vi "Measurement UI.vi"() -> ()   [LabVIEW 2025, in "I2C Bus Monitor UI.lvlib"]
uses:
  I2C Bus Monitor UI.lvlib
  OOB gRPC Client/RPC Messages/hwval_GenericRequest.ctl
  042a6803-d82a-4003-9d1e-a547103779a0.vi
  SubVIs/Table Buffer - Check.vi
  SubVIs/Table Buffer - Create.vi
  SubVIs/Table Buffer - Destroy.vi
  OOB gRPC Client/OOB gRPC Client.lvlib
panel:
  in  "HELP":bool
  in  "CMPLX SCRIPT":bool
  out "RUNNING":bool
  in  "Monitor Tab":enum32{"Monitor", "Scan"}(tab)
  out "# TXNS IN TABLE":i32
  in  "PauseResume":bool=TRUE
  out "STREAMING":bool
  in  "CSV FILE PATH":path
  in  "Save CSV":bool
  out "# TXNS IN BUFFER":i32
  in  "Clear":bool
  out "MONITOR TABLE":string[][](table)
  in  "Scan Bus":bool
  out "Scan Table":string[][](table)
  out "BUSY":bool
  in  "Debug&Hidden":enum32{"Debug", "Hidden"}(tab)
  out "Message Buffer Pressure (Logic)":i32
  out "Transactions in Buffer (UI)":i32
  out "FIFO Overflow":bool
  out "FIFO Pressure":u32
  out "Measurement Logic Counter":i32
  out "FIFO Msg Fetch Count":i32
  out "OOB gRPC Port":i32
  in  "Bitfile Path":string
  in  "Alias Name":string
  in  "Serial Input":string
  out "Error (Logic)":string
  out "Scanned Addresses":i32[](array[numeric]) format="%.0x"
  out "Status":string
  in  "Send I2C CMD":bool
  in  "R/W":bool
  in  "DATA":u8 format="%02x"
  in  "REG. ADDR.":u16 format="%04x"
  in  "SLAVE ADDR.":u8 format="%02x"
  in  "Send I2C Script":bool
  in  "CONFIG SCRIPT FILE PATH":path
  in  "SERIAL INPUT (SI)":u32(ring)
  in  "RESOURCE NAME":u32(ring)
  # "NOTE:\nFlat Box sizes are specifically chosen to fit into IS small panel without a horizontal scrollbar"
  # "CONFIGURATION"
  # "I2C TRANSACTIONS"
  # "I2C MONITOR"
  # "STATUS"
  # "These controls are mainly used to transfer data from logic to ui via configs/results, but don't need to be visible."
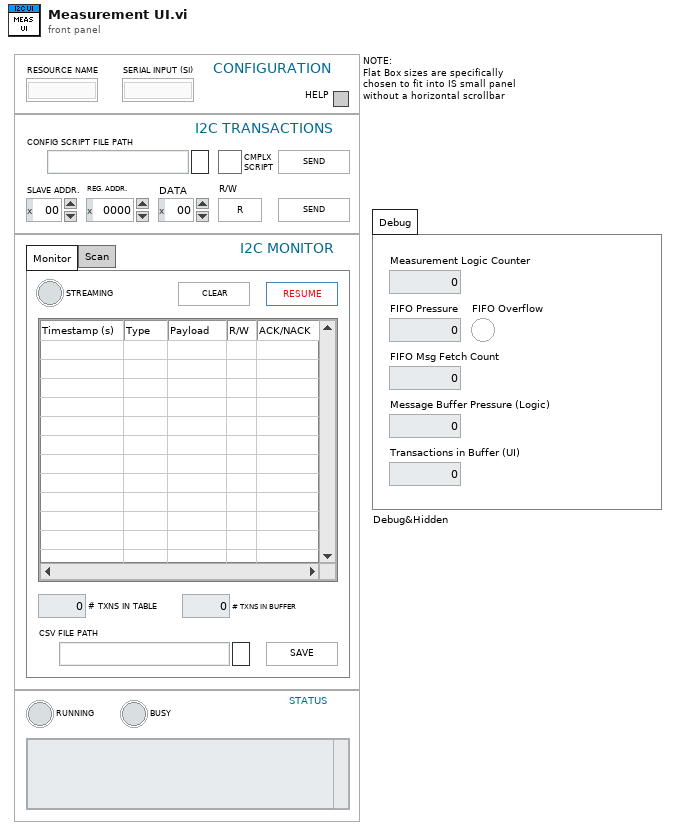
[diagram p1: front panel]
types:
  T1 = cluster{"Measurement Logic Counter":refnum<vi>, "OOB gRPC Port":refnum<vi>, "Bitfile Path":refnum<vi>, "RESOURCE NAME":refnum<vi>, "Alias Name":refnum<vi>, "SERIAL INPUT (SI)":refnum<vi>, "Serial Input":refnum<vi>, "MONITOR TABLE":refnum<vi>, "FIFO Msg Fetch Count":refnum<vi>, "STREAMING":refnum<vi>, "PauseResume":refnum<vi>, "Transactions in Buffer (UI)":refnum<vi>, "CSV FILE PATH":refnum<vi>, "BUSY":refnum<vi>, "Status":refnum<vi>, "Error (Logic)":refnum<vi>, "Scan Table":refnum<vi>, "Scanned Addresses":refnum<vi>, "# TXNS IN BUFFER":refnum<vi>, "# TXNS IN TABLE":refnum<vi>, "RUNNING":refnum<vi>}
  T2 = typedef "OOB gRPC Client.lvlib/hwval_GenericRequest.ctl" = cluster{"Command":string, "Payload":u8[]}
  T3 = typedef "OOB gRPC Client.lvlib/hwval_GenericResponse.ctl" = cluster{"Payload":u8[]}
  T4 = typedef "grpc-lvsupport-release.lvlib/grpcId.ctl" = u64
  T5 = cluster{"NewVal":bool, string, "CMPLX SCRIPT":bool}
  T6 = cluster{"NewVal":bool, "SLAVE ADDR.":u8, "REG. ADDR.":u16, "DATA":u8, "R/W":bool}
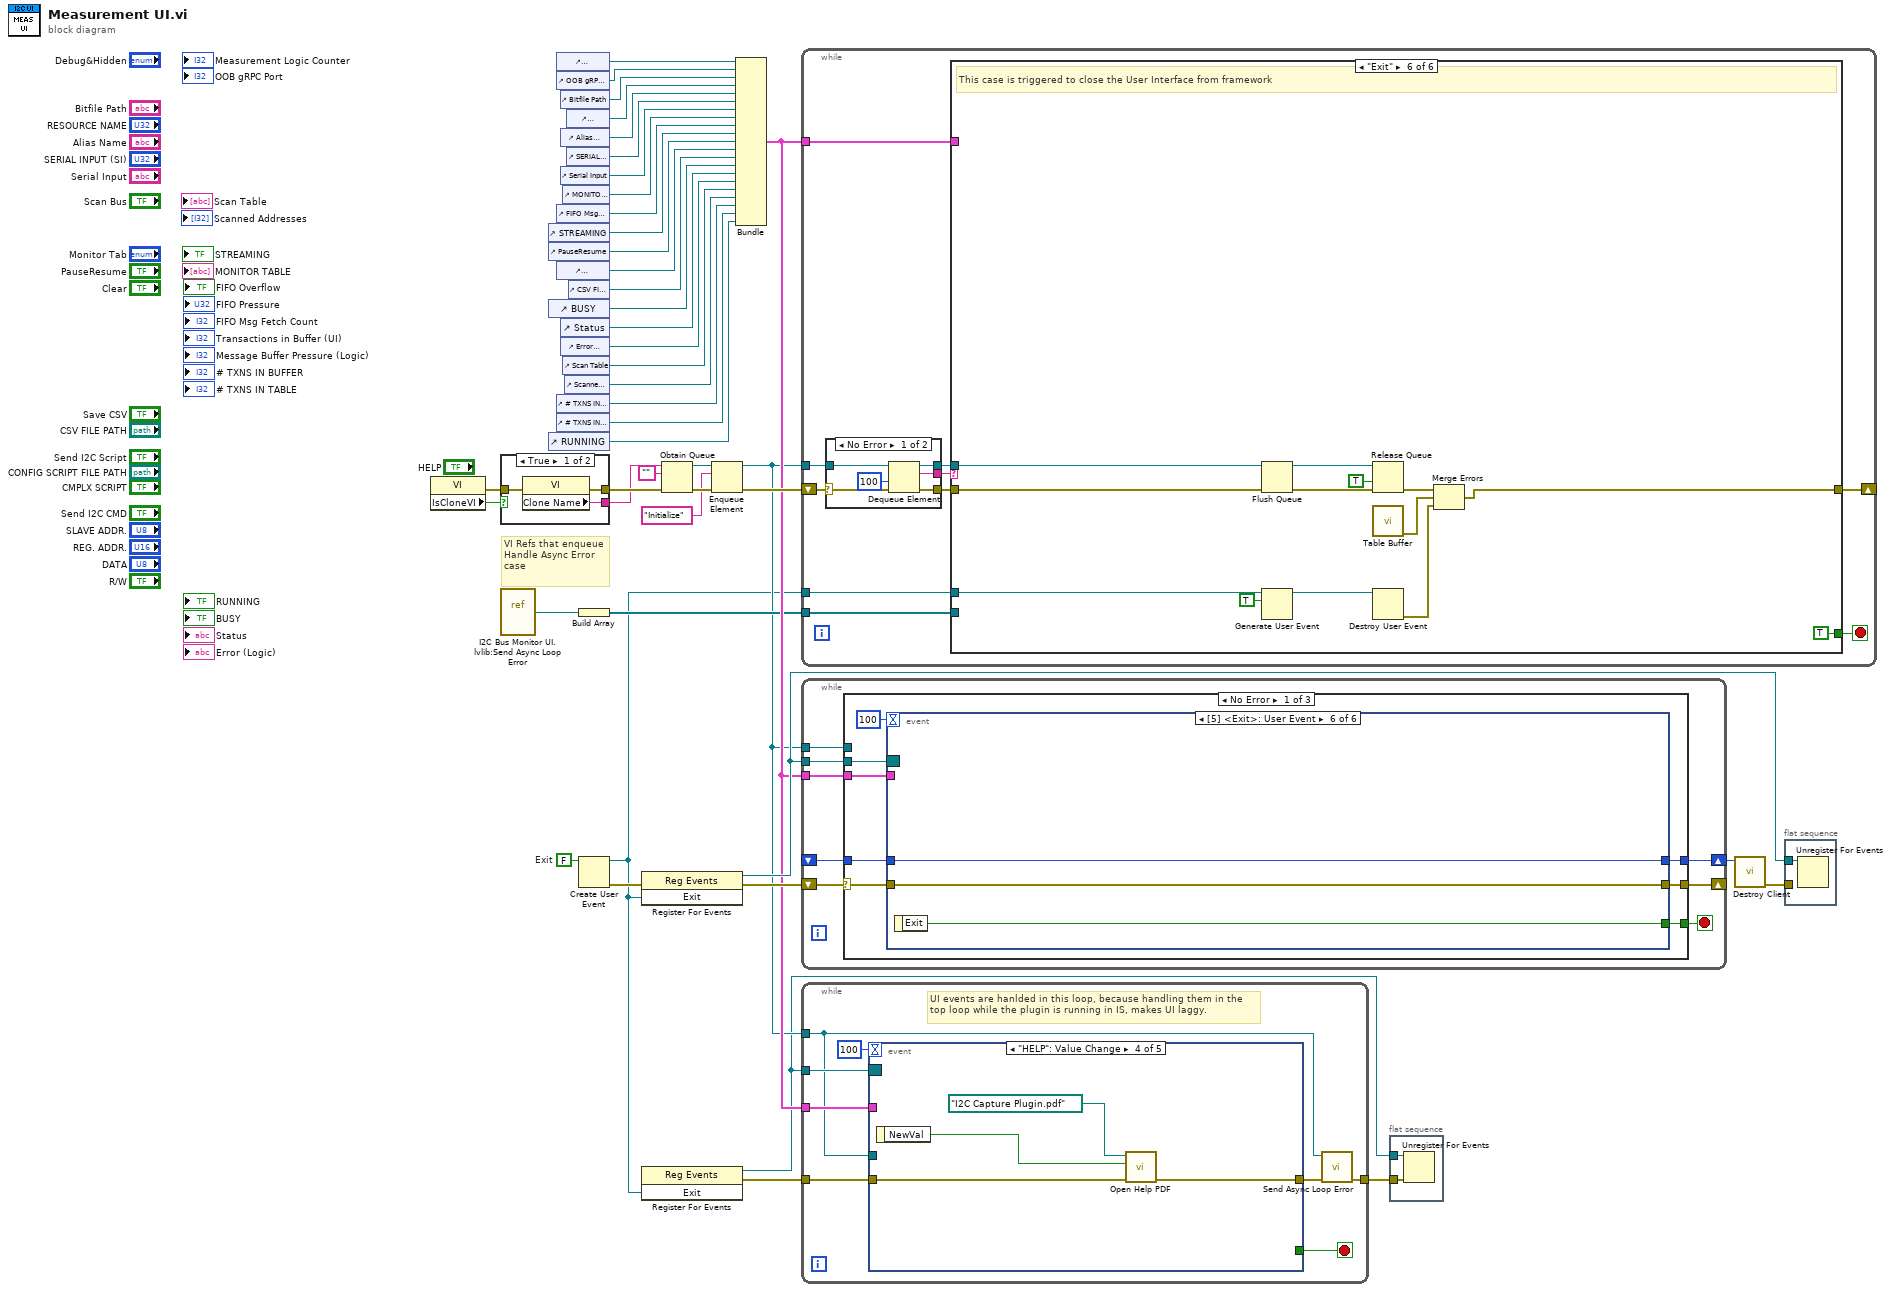
[diagram p0: block diagram]
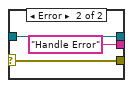
[diagram p2: hidden frame]
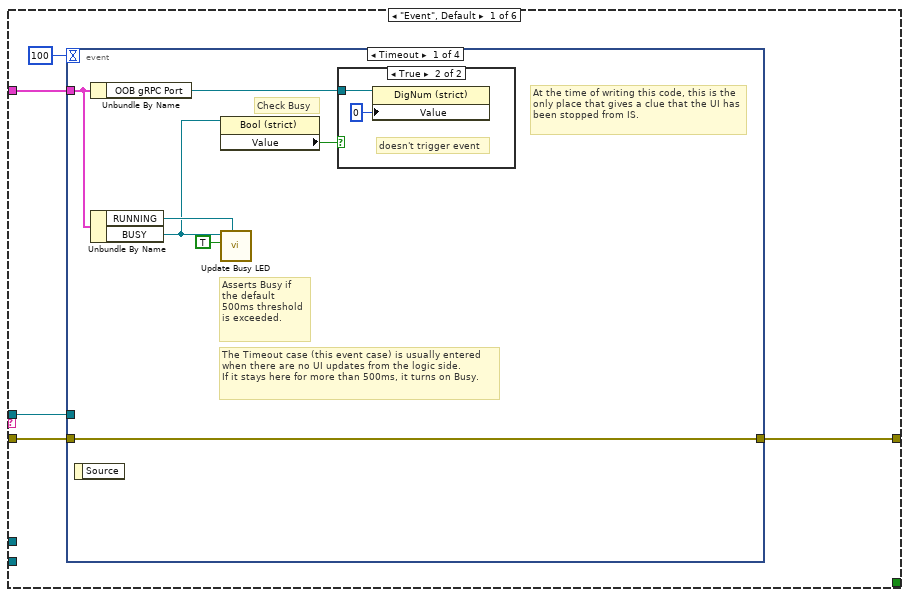
[diagram p3: hidden frame]
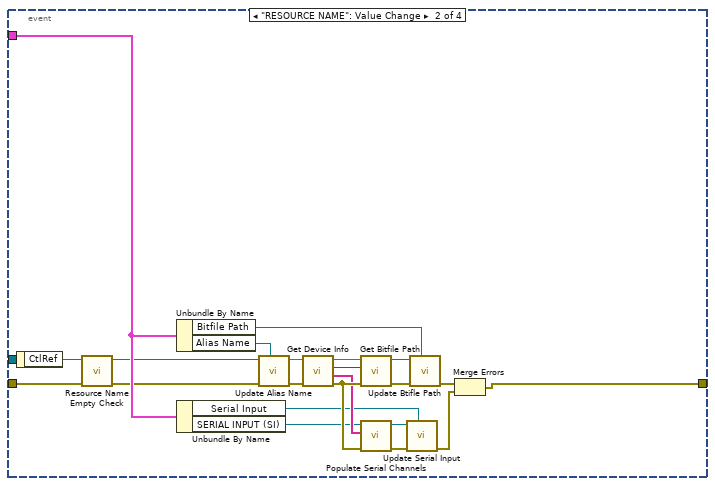
[diagram p5: hidden frame]
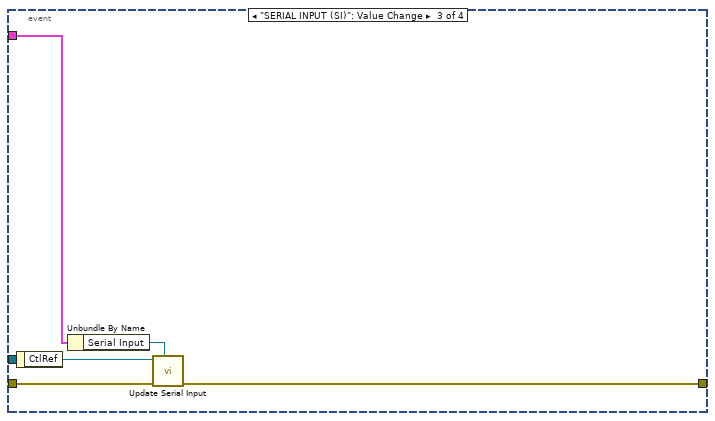
[diagram p6: hidden frame]
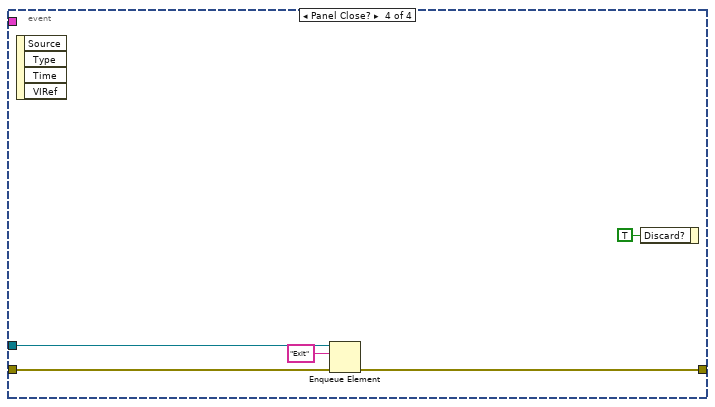
[diagram p7: hidden frame]
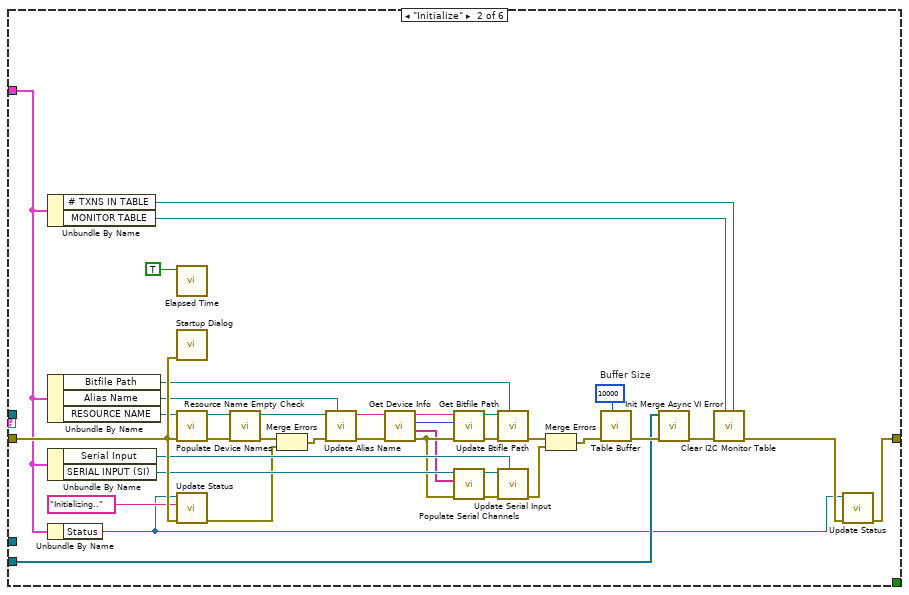
[diagram p8: hidden frame]
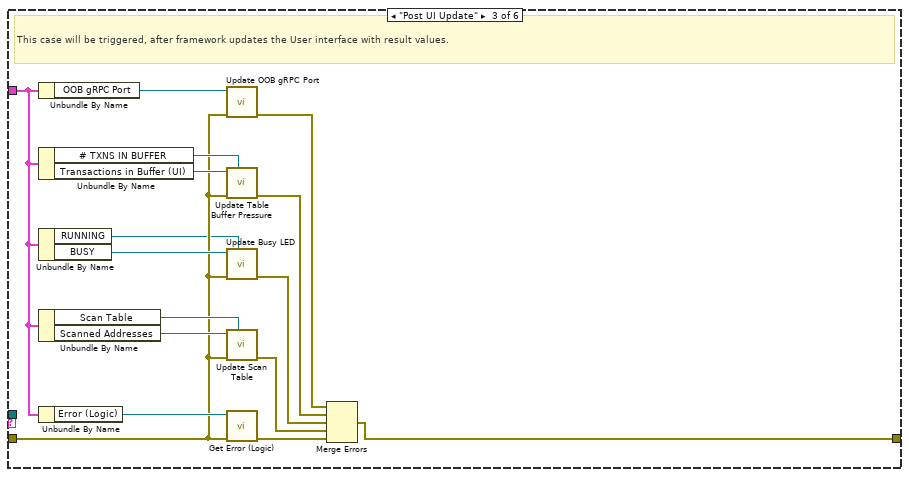
[diagram p9: hidden frame]
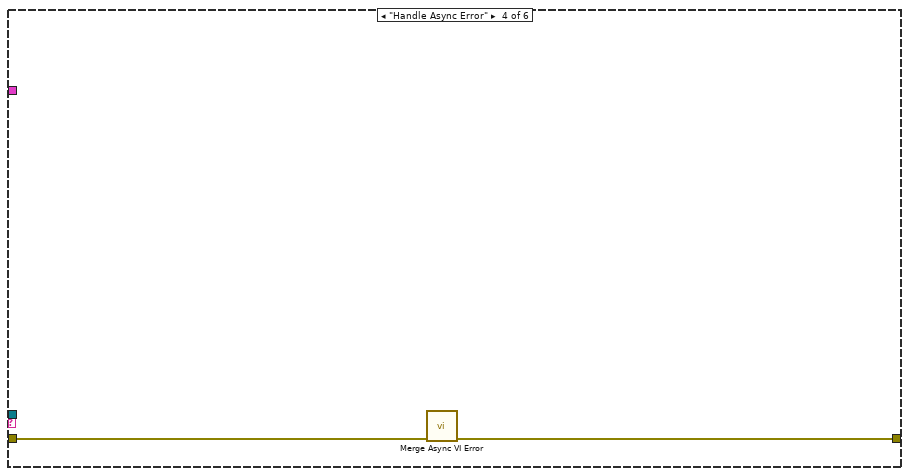
[diagram p10: hidden frame]
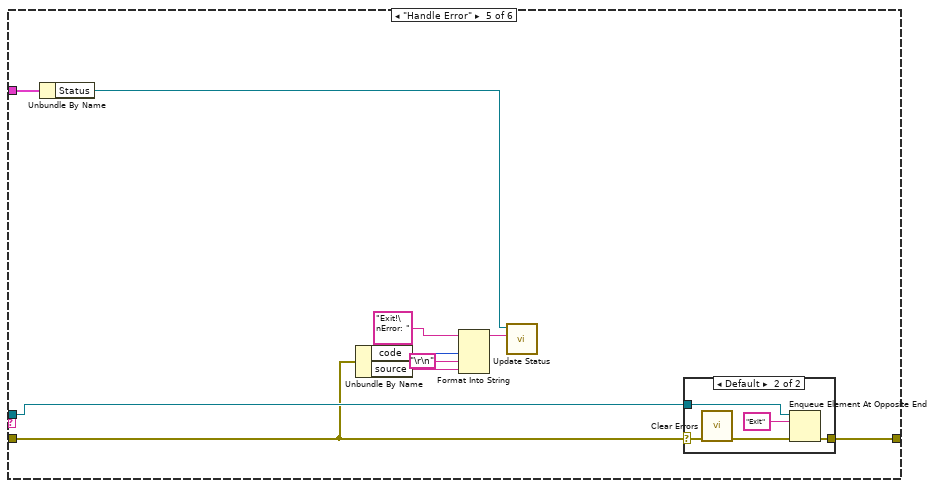
[diagram p11: hidden frame]
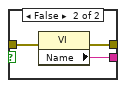
[diagram p13: hidden frame]
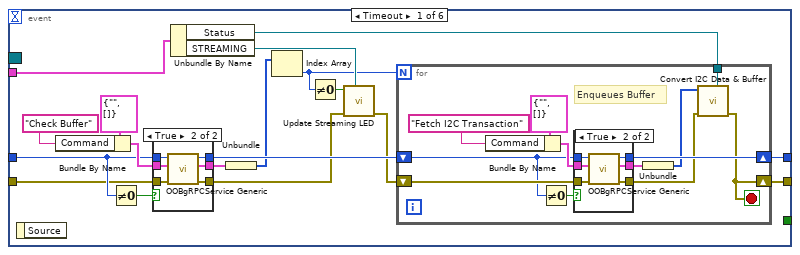
[diagram p14: hidden frame]
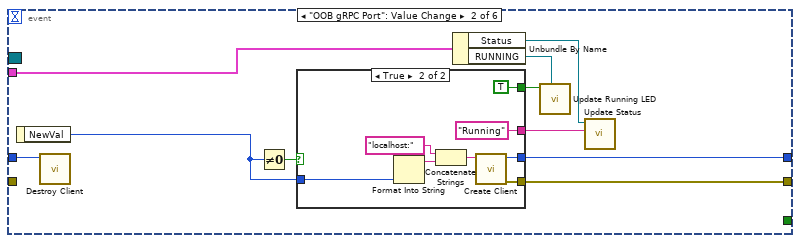
[diagram p17: hidden frame]
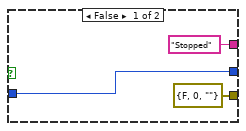
[diagram p18: hidden frame]
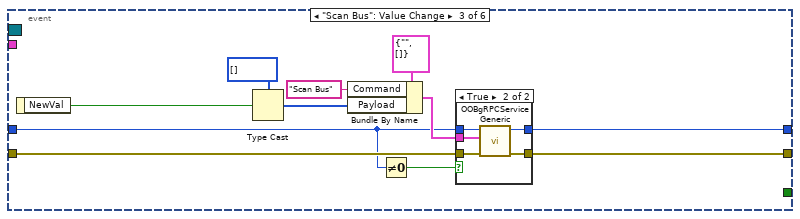
[diagram p19: hidden frame]
diagram:
  w35 = FALSE  # Exit
  # "VI Refs that enqueue Handle Async Error case"
  n1 = property class="VI"() -> (error out=w32:errorcluster, "IsCloneVI"=w36:bool)  [unwired: 2 in, 1 out]
  n2 = case shown="True" w36 {
    tunnel: [w47 w50] -> w43
    tunnel: [w46 w49] -> w42
    tunnel: w32 -> [w45 w48]
    frame True {
      n3 = property class="VI"(error in=w45) -> (error out=w47:errorcluster, "Clone Name"=w46:string)  [unwired: 1 in, 1 out]
    }
    frame False {
      n4 = property class="VI"(error in=w48) -> (error out=w50:errorcluster, "Name"=w49:string)  [unwired: 1 in, 1 out]
    }
  }
  n5 = vi-ref "I2C Bus Monitor UI.lvlib:Send Async Loop Error.vi"() -> (w6:refnum<vi>)
  n6 = control-ref of="STREAMING"() -> (w19:refnum<vi>)
  n7 = control-ref of="PauseResume"() -> (w24:refnum<vi>)
  n8 = control-ref of="BUSY"() -> (w17:refnum<vi>)
  n9 = control-ref of="RUNNING"() -> (w8:refnum<vi>)
  n10 = control-ref of="Measurement Logic Counter"() -> (w18:refnum<vi>)
  n11 = control-ref of="OOB gRPC Port"() -> (w30:refnum<vi>)
  n12 = control-ref of="FIFO Msg Fetch Count"() -> (w31:refnum<vi>)
  n13 = control-ref of="Transactions in Buffer (UI)"() -> (w23:refnum<vi>)
  n14 = control-ref of="# TXNS IN BUFFER"() -> (w10:refnum<vi>)
  n15 = control-ref of="# TXNS IN TABLE"() -> (w9:refnum<vi>)
  n16 = control-ref of="Bitfile Path"() -> (w25:refnum<vi>)
  n17 = control-ref of="Alias Name"() -> (w27:refnum<vi>)
  n18 = control-ref of="Serial Input"() -> (w29:refnum<vi>)
  n19 = control-ref of="Status"() -> (w15:refnum<vi>)
  n20 = control-ref of="Error (Logic)"() -> (w14:refnum<vi>)
  n21 = control-ref of="MONITOR TABLE"() -> (w21:refnum<vi>)
  n22 = control-ref of="Scan Table"() -> (w12:refnum<vi>)
  n23 = control-ref of="Scanned Addresses"() -> (w11:refnum<vi>)
  n24 = control-ref of="RESOURCE NAME"() -> (w26:refnum<vi>)
  n25 = control-ref of="SERIAL INPUT (SI)"() -> (w28:refnum<vi>)
  n26 = control-ref of="CSV FILE PATH"() -> (w22:refnum<vi>)
  n27 = Build Array(w6) -> (w13:refnum<vi>[])
  n28 = Create User Event(user event datatype=w35) -> (user event=w1:refnum<user-event>, error out=w34:errorcluster)  [unwired: 1 in]
  n29 = register-events(error in=w34, w1) -> (reference out=w20:refnum<event-registration>, error out=w44:errorcluster)  [unwired: 1 in]
  n30 = register-events(w1) -> (reference out=w3:refnum<event-registration>, error out=w2:errorcluster)  [unwired: 2 in]
  n31 = Obtain Queue(name (unnamed)=w42, element data type="", error in (no error)=w43) -> (queue out=w39:refnum<queue>, error out=w41:errorcluster)  [unwired: 2 in, 1 out]
  n32 = Enqueue Element(queue=w39, element="Initialize", error in (no error)=w41) -> (queue out=w7:refnum<queue>, error out=w40:errorcluster)  [unwired: 1 in, 1 out]
  n33 = Bundle("Measurement Logic Counter"=w18, "OOB gRPC Port"=w30, "Bitfile Path"=w25, "RESOURCE NAME"=w26, "Alias Name"=w27, "SERIAL INPUT (SI)"=w28, "Serial Input"=w29, "MONITOR TABLE"=w21, "FIFO Msg Fetch Count"=w31, "STREAMING"=w19, "PauseResume"=w24, "Transactions in Buffer (UI)"=w23, "CSV FILE PATH"=w22, "BUSY"=w17, "Status"=w15, "Error (Logic)"=w14, "Scan Table"=w12, "Scanned Addresses"=w11, "# TXNS IN BUFFER"=w10, "# TXNS IN TABLE"=w9, "RUNNING"=w8) -> (w16:T1)  [unwired: 1 in]
  n34 = while {
    shift-right: [w55] -> _
    shift-left: w40 -> [w60]
    tunnel: w7 -> [w58]
    tunnel: w1 -> [w53]
    tunnel: w16 -> [w52]
    tunnel: w13 -> [w51]
    stop <- w54 stop-if-true
    n35 = case shown="No Error" w60 {
      selector: w60 -> [w66 w69]
      tunnel: [w65 w69] -> w59
      tunnel: w58 -> [w64 w68]
      tunnel: [w63 w68] -> w57
      tunnel: [w62 "Handle Error"] -> w56
      frame No Error {
        n36 = Dequeue Element(queue=w64, timeout in ms (-1)=100, error in (no error)=w66) -> (queue out=w63:refnum<queue>, element=w62:string, error out=w65:errorcluster)  [unwired: 1 out]
      }
      frame Error {
      }
    }
    n37 = case shown="\"Exit\"" w56 {
      tunnel: w59 -> [w73 w151 w154 w170 w175 w192]
      tunnel: w57 -> [w71 _ _ _ w176 w198]
      tunnel: [w74 w116 w167 w169 w174 w191] -> w55
      tunnel: [_ _ _ _ _ TRUE] -> w54
      tunnel: w53 -> [_ _ _ _ _ w193]
      tunnel: w52 -> [w70 w120 w160 _ w172 _]
      tunnel: w51 -> [_ w143 _ _ _ _]
      frame "Event", Default {
        n38 = event shown="[0] Timeout" {
          selector: _ -> [_ _ _ _]
          dyn-events: _ -> [_ _ _ _]
          timeout: 100 -> [_ _ _ _]
          tunnel: [w81 w100 w106 w113] -> w74
          tunnel: w73 -> [w81 w96 w110 w114]
          tunnel: w71 -> [_ _ _ w112]
          tunnel: w70 -> [w79 w98 w108 _]
          event Timeout {
            # "The Timeout case (this event case) is usually entered when there are no UI updates from the logic side. \nIf it stays here for more than 500ms, it turns on Busy."
            # "Asserts Busy if the default 500ms threshold is exceeded."
            # "Check Busy"
            # "At the time of writing this code, this is the only place that gives a clue that the UI has been stopped from IS."
            n39 = event-data() -> ()  [unwired: 1 in, 1 out]
            n40 = Unbundle By Name(w79) -> ("OOB gRPC Port"=w80:refnum<vi>)
            n41 = Unbundle By Name(w79) -> ("RUNNING"=w77:refnum<vi>, "BUSY"=w76:refnum<vi>)
            n42 = property on="Property Node" class="Bool (strict)"(reference=w76) -> ("Value"=w75:bool)  [unwired: 1 in, 2 out]
            n43 = call "Update Busy LED.vi"("RUNNING Ref"=w77, "Busy (False)"=TRUE ("value"), "BUSY Ref"=w76) -> ()  [unwired: 8 in, 1 out]
            n44 = case shown="True" w75 {
              tunnel: w80 -> [_ w83]
              frame False {
              }
              frame True {
                # "doesn't trigger event"
                n45 = property on="Property Node" class="DigNum (strict)"(reference=w83, "Value"=0 ("OOB gRPC Port")) -> ()  [unwired: 1 in, 2 out]
              }
            }
          }
          event "RESOURCE NAME": Value Change {
            n46 = event-data() -> ("CtlRef"=w85:refnum<vi>)  [unwired: 1 in]
            n47 = call "Resource Name Empty Check.vi"("error in (no error)"=w96, "RESOURCE NAME Ref"=w85) -> ("error out"=w86:errorcluster, "RESOURCE NAME Ref out"=w84:refnum<vi>)  [unwired: 8 in]
            n48 = Unbundle By Name(w98) -> ("Bitfile Path"=w88:refnum<vi>, "Alias Name"=w93:refnum<vi>)
            n49 = Unbundle By Name(w98) -> ("Serial Input"=w90:refnum<vi>, "SERIAL INPUT (SI)"=w97:refnum<vi>)
            n50 = call "Update Alias Name.vi"("Alias Name Ref"=w93, "error in (no error)"=w86, "RESOURCE NAME Ref"=w84) -> ("error out"=w94:errorcluster, "Alias Name"=w95:string)  [unwired: 7 in]
            n51 = call "Get Device Info.vi"("error in (no error)"=w94, "RIO Device"=w95) -> ("error out"=w105:errorcluster, "SI Channels"=w102:string[], "SI Count"=w104:i32, "Module Name"=w103:string)  [unwired: 6 in]
            n52 = call "Get Bitfile Path.vi"("error in (no error)"=w105, "SI Count"=w104, "Module Name"=w103) -> ("error out"=w101:errorcluster, "Bitfile Path"=w87:path)  [unwired: 7 in]
            n53 = call "Populate Serial Channels.vi"("error in (no error)"=w105, "Strings []"=w102, "SERIAL INPUT (SI) Ref in"=w97) -> ("error out"=w99:errorcluster, "SERIAL INPUT (SI) Ref out"=w91:refnum<vi>)  [unwired: 7 in]
            n54 = call "Update Serial Input.vi"("Serial Input Ref"=w90, "error in (no error)"=w99, "SERIAL INPUT (SI) Ref"=w91) -> ("error out"=w92:errorcluster)  [unwired: 8 in]
            n55 = call "Update Btifle Path.vi"("Bitfile Path Ref"=w88, "error in (no error)"=w101, "Bitfile Path"=w87) -> ("error out"=w89:errorcluster)  [unwired: 8 in]
            n56 = Merge Errors(w89, w92) -> (w100:errorcluster)
          }
          event "SERIAL INPUT (SI)": Value Change {
            n57 = event-data() -> ("CtlRef"=w109:refnum<vi>)  [unwired: 1 in]
            n58 = Unbundle By Name(w108) -> ("Serial Input"=w107:refnum<vi>)
            n59 = call "Update Serial Input.vi"("Serial Input Ref"=w107, "error in (no error)"=w110, "SERIAL INPUT (SI) Ref"=w109) -> ("error out"=w106:errorcluster)  [unwired: 8 in]
          }
          event Panel Close? {
            n60 = event-data() -> ()  [unwired: 1 in, 4 out]
            n61 = Enqueue Element(queue=w112, element="Exit", error in (no error)=w114) -> (error out=w113:errorcluster)  [unwired: 1 in, 2 out]
            n62 = event-data("Discard?"=TRUE) -> ()  [unwired: 1 in, 1 out]
          }
        }
      }
      frame "Initialize" {
        w142 = 10000  # Buffer Size
        n63 = Unbundle By Name(w120) -> ("# TXNS IN TABLE"=w119:refnum<vi>, "MONITOR TABLE"=w118:refnum<vi>)
        n64 = Unbundle By Name(w120) -> ("Bitfile Path"=w146:refnum<vi>, "Alias Name"=w148:refnum<vi>, "RESOURCE NAME"=w150:refnum<vi>)
        n65 = Unbundle By Name(w120) -> ("Serial Input"=w147:refnum<vi>, "SERIAL INPUT (SI)"=w149:refnum<vi>)
        n66 = Unbundle By Name(w120) -> ("Status"=w121:refnum<vi>)
        n67 = call "Elapsed Time.vi"("Reset"=TRUE) -> ()  [unwired: 9 in, 2 out]
        n68 = call "Startup Dialog.vi"("error in"=w151) -> ()  [unwired: 10 in, 1 out]
        n69 = call "Populate Device Names.vi"("error in (no error)"=w151, "RESOURCE NAME Ref"=w150) -> ("error out"=w123:errorcluster, "RESOURCE NAME Ref out"=w140:refnum<vi>)  [unwired: 8 in]
        n70 = call "Update Status.vi"("error in (no error)"=w151, "Value"="Initializing..", "Status Ref"=w121) -> ("error out"=w136:errorcluster)  [unwired: 8 in]
        n71 = call "Resource Name Empty Check.vi"("error in (no error)"=w123, "RESOURCE NAME Ref"=w140) -> ("error out"=w122:errorcluster, "RESOURCE NAME Ref out"=w139:refnum<vi>)  [unwired: 8 in]
        n72 = Merge Errors(w122, w136) -> (w138:errorcluster)
        n73 = call "Update Alias Name.vi"("Alias Name Ref"=w148, "error in (no error)"=w138, "RESOURCE NAME Ref"=w139) -> ("error out"=w129:errorcluster, "Alias Name"=w128:string)  [unwired: 7 in]
        n74 = call "Get Device Info.vi"("error in (no error)"=w129, "RIO Device"=w128) -> ("error out"=w135:errorcluster, "SI Channels"=w132:string[], "SI Count"=w134:i32, "Module Name"=w133:string)  [unwired: 6 in]
        n75 = call "Get Bitfile Path.vi"("error in (no error)"=w135, "SI Count"=w134, "Module Name"=w133) -> ("error out"=w131:errorcluster, "Bitfile Path"=w124:path)  [unwired: 7 in]
        n76 = call "Populate Serial Channels.vi"("error in (no error)"=w135, "Strings []"=w132, "SERIAL INPUT (SI) Ref in"=w149) -> ("error out"=w130:errorcluster, "SERIAL INPUT (SI) Ref out"=w126:refnum<vi>)  [unwired: 7 in]
        n77 = call "Update Btifle Path.vi"("Bitfile Path Ref"=w146, "error in (no error)"=w131, "Bitfile Path"=w124) -> ("error out"=w125:errorcluster)  [unwired: 8 in]
        n78 = call "Update Serial Input.vi"("Serial Input Ref"=w147, "error in (no error)"=w130, "SERIAL INPUT (SI) Ref"=w126) -> ("error out"=w127:errorcluster)  [unwired: 8 in]
        n79 = Merge Errors(w125, w127) -> (w137:errorcluster)
        n80 = call-poly "Table Buffer.vi"("Buffer Size (10k)"=w142, "error in (no error)"=w137) -> ("error out"=w145:errorcluster)  [unwired: 9 in]
        n81 = call "Init Merge Async VI Error.vi"("error in (no error)"=w145, "VI Ref"=w143) -> ("error out"=w117:errorcluster)  [unwired: 9 in]
        n82 = call "Clear I2C Monitor Table.vi"("# TXNS IN TABLE Ref"=w119, "I2C Table Ref"=w118, "error in (no error)"=w117) -> ("error out"=w152:errorcluster)  [unwired: 8 in]
        n83 = call "Update Status.vi"("error in (no error)"=w152, "Status Ref"=w121) -> ("error out"=w116:errorcluster)  [unwired: 9 in]
      }
      frame "Post UI Update" {
        # "This case will be triggered, after framework updates the User interface with result values."
        n84 = Unbundle By Name(w160) -> ("OOB gRPC Port"=w168:refnum<vi>)
        n85 = Unbundle By Name(w160) -> ("# TXNS IN BUFFER"=w157:refnum<vi>, "Transactions in Buffer (UI)"=w165:refnum<vi>)
        n86 = Unbundle By Name(w160) -> ("RUNNING"=w153:refnum<vi>, "BUSY"=w162:refnum<vi>)
        n87 = Unbundle By Name(w160) -> ("Scan Table"=w159:refnum<vi>, "Scanned Addresses"=w158:refnum<vi>)
        n88 = Unbundle By Name(w160) -> ("Error (Logic)"=w161:refnum<vi>)
        n89 = call "Update OOB gRPC Port.vi"("error in (no error)"=w154, "OOB gRPC Port Ref in"=w168) -> ("error out"=w166:errorcluster)  [unwired: 9 in]
        n90 = call "Update Table Buffer Pressure.vi"("BUFFER Ref"=w157, "error in (no error)"=w154, "Table Buffer Pressure Ref"=w165) -> ("error out"=w164:errorcluster)  [unwired: 8 in]
        n91 = call "Update Busy LED.vi"("RUNNING Ref"=w153, "error in (no error)"=w154, "BUSY Ref"=w162) -> ("error out"=w163:errorcluster)  [unwired: 8 in]
        n92 = call "Update Scan Table.vi"("Scan Table Ref"=w159, "error in (no error)"=w154, "Scanned Addresses Ref"=w158) -> ("error out"=w155:errorcluster)  [unwired: 8 in]
        n93 = call "Get Error (Logic).vi"("error in (no error)"=w154, "Error (Logic)Ref"=w161) -> ("error out"=w156:errorcluster)  [unwired: 9 in]
        n94 = Merge Errors(w166, w164, w163, w155, w156) -> (w167:errorcluster)
      }
      frame "Handle Async Error" {
        n95 = call "Merge Async VI Error.vi"("error in (no error)"=w170) -> ("error out"=w169:errorcluster)  [unwired: 10 in]
      }
      frame "Handle Error" {
        n96 = Unbundle By Name(w172) -> ("Status"=w173:refnum<vi>)
        n97 = Unbundle By Name(w175) -> ("code"=w180:i32, "source"=w179:string)
        n98 = Format Into String(initial string="Exit!\nError: " ("format string"), w180, "\r\n", w179) -> (resulting string=w171:string)  [unwired: 2 in, 1 out]
        n99 = call "Update Status.vi"("Value"=w171, "Status Ref"=w173) -> ()  [unwired: 9 in, 1 out]
        n100 = case shown="Default" w175 {
          selector: w175 -> [w181 w186]
          tunnel: [w181 w185] -> w174
          tunnel: w176 -> [_ w183]
          frame No Error {
          }
          frame Default {
            n101 = call <vilib>:"Clear Errors.vi"("error in (no error)"=w186) -> ("error out"=w184:errorcluster)  [unwired: 5 in, 1 out]
            n102 = Enqueue Element At Opposite End(queue=w183, element="Exit", error in (no error)=w184) -> (error out=w185:errorcluster)  [unwired: 1 in, 2 out]
          }
        }
      }
      frame "Exit" {
        # "This case is triggered to close the User Interface from framework"
        n103 = Flush Queue(queue=w198, error in (no error)=w192) -> (queue out=w197:refnum<queue>, error out=w196:errorcluster)  [unwired: 1 out]
        n104 = Generate User Event(user event=w193, event data cluster=TRUE ("event data")) -> (user event out=w188:refnum<user-event>)  [unwired: 2 in, 1 out]
        n105 = Release Queue(queue=w197, force destroy? (F)=TRUE, error in (no error)=w196) -> (error out=w195:errorcluster)  [unwired: 2 out]
        n106 = call-poly "Table Buffer.vi"() -> ("error out"=w189:errorcluster)  [unwired: 11 in]
        n107 = Destroy User Event(user event=w188) -> (error out=w190:errorcluster)  [unwired: 1 in]
        n108 = Merge Errors(w195, w189, w190) -> (w191:errorcluster)
      }
    }
  }
  n109 = while {
    tunnel: w20 -> [w204]
    shift-right: [w205] -> _
    shift-left: w44 -> [w207]
    shift-right: [w202] -> w33
    shift-left: _ -> [w203]
    tunnel: w16 -> [w201]
    tunnel: w7 -> [w200]
    stop <- w206 stop-if-true
    n110 = case shown="No Error" w207 {
      selector: w207 -> [w213 w354 _]
      tunnel: [w210 TRUE w364] -> w206
      tunnel: [w214 w352 errorcluster {"status"=FALSE, "code"=0, "source"=""} ("error IO")] -> w205
      tunnel: w204 -> [w215 _ _]
      tunnel: w203 -> [w212 w355 w363]
      tunnel: [w211 w355 w363] -> w202
      tunnel: w201 -> [w208 _ w358]
      tunnel: w200 -> [_ w353 _]
      frame No Error {
        n111 = event shown="[5] <Exit>: User Event" {
          selector: w215 -> [_ _ _ _ _ _]
          dyn-events: _ -> [_ _ _ _ _ _]
          timeout: 100 -> [_ _ _ _ _ _]
          tunnel: [w217 w271 w286 w311 w335 w348] -> w214
          tunnel: w213 -> [w225 _ w285 w303 w329 w348]
          tunnel: w212 -> [w226 w270 w284 w310 w334 w349]
          tunnel: [w232 w269 w287 w312 w336 w349] -> w211
          tunnel: [_ _ _ _ _ w350] -> w210
          tunnel: w208 -> [w218 w266 _ _ _ _]
          event Timeout {
            n112 = event-data() -> ()  [unwired: 1 in, 1 out]
            n113 = Bundle By Name(cluster=T2 {"Command"="", "Payload"=[]} ("Request Data"), "Command"="Check Buffer") -> (w229:T2)
            n114 = Not Equal To 0?(x=w226) -> (x != 0?=w228:bool)
            n115 = case shown="True" w228 {
              tunnel: [w255 w258] -> w224
              tunnel: [w254 w257] -> w222
              tunnel: w226 -> [w255 w261]
              tunnel: w225 -> [w254 w260]
              tunnel: w229 -> [_ w259]
              tunnel: [_ w256] -> w231
              frame False {
              }
              frame True {
                n116 = call "OOBgRPCService Generic.vi"("error in"=w260, "Request Data"=w259, "gRPC ID"=w261) -> ("error out"=w257:errorcluster, "Response Data"=w256:T3, "gRPC ID out"=w258:T4)  [unwired: 6 in]
              }
            }
            n117 = Unbundle By Name(w218) -> ("Status"=w216:refnum<vi>, "STREAMING"=w233:refnum<vi>)
            n118 = Unbundle(w231) -> ("Payload"=w223:u8[])
            n119 = Index Array(array=w223) -> (element=w219:u8)  [unwired: 1 in]
            n120 = Not Equal To 0?(x=w219) -> (x != 0?=w220:bool)
            n121 = call "Update Streaming LED.vi"("STREAMING Ref"=w233, "error in (no error)"=w222, "Value"=w220) -> ("error out"=w221:errorcluster)  [unwired: 8 in]
            n122 = for {
              N: w219 -> [_]
              shift-right: [w236] -> w217
              shift-left: w221 -> [w245]
              shift-right: [w240] -> w232
              shift-left: w224 -> [w237]
              tunnel: w216 -> [w234]
              stop <- w236 stop-if-true
              # "Enqueues Buffer"
              n123 = Bundle By Name(cluster=T2 {"Command"="", "Payload"=[]} ("Request Data"), "Command"="Fetch I2C Transaction") -> (w243:T2)
              n124 = Not Equal To 0?(x=w237) -> (x != 0?=w244:bool)
              n125 = case shown="True" w244 {
                tunnel: [w247 w250] -> w240
                tunnel: [w246 w249] -> w238
                tunnel: w237 -> [w247 w253]
                tunnel: w245 -> [w246 w252]
                tunnel: w243 -> [_ w251]
                tunnel: [_ w248] -> w239
                frame False {
                }
                frame True {
                  n126 = call "OOBgRPCService Generic.vi"("error in"=w252, "Request Data"=w251, "gRPC ID"=w253) -> ("error out"=w249:errorcluster, "Response Data"=w248:T3, "gRPC ID out"=w250:T4)  [unwired: 6 in]
                }
              }
              n127 = Unbundle(w239) -> ("Payload"=w235:u8[])
              n128 = call "Convert I2C Data & Buffer.vi"("Status Ref"=w234, "error in (no error)"=w238, "Data"=w235) -> ("error out"=w236:errorcluster)  [unwired: 8 in]
            }
          }
          event "OOB gRPC Port": Value Change {
            n129 = event-data() -> ("NewVal"=w267:i32)  [unwired: 1 in]
            n130 = call "Destroy Client.vi"("gRPC ID"=w270) -> ()  [unwired: 10 in, 1 out]
            n131 = Not Equal To 0?(x=w267) -> (x != 0?=w268:bool)
            n132 = case shown="True" w268 {
              tunnel: [errorcluster {"status"=FALSE, "code"=0, "source"=""} ("error out") w282] -> w271
              tunnel: w267 -> [w274 w278]
              tunnel: [w274 w277] -> w269
              tunnel: [_ TRUE ("Value")] -> w264
              tunnel: ["Stopped" ("Value") "Running" ("Value")] -> w262
              frame False {
              }
              frame True {
                n133 = Format Into String(w278) -> (resulting string=w281:string)  [unwired: 3 in, 1 out]
                n134 = Concatenate Strings("localhost:" ("string"), w281) -> (w279:string)
                n135 = call "Create Client.vi"("address"=w279) -> ("error out"=w282:errorcluster, "gRPC ID Out"=w277:T4)  [unwired: 9 in]
              }
            }
            n136 = Unbundle By Name(w266) -> ("Status"=w263:refnum<vi>, "RUNNING"=w265:refnum<vi>)
            n137 = call "Update Running LED.vi"("RUNNING Ref"=w265, "Value"=w264) -> ()  [unwired: 9 in, 1 out]
            n138 = call "Update Status.vi"("Value"=w262, "Status Ref"=w263) -> ()  [unwired: 9 in, 1 out]
          }
          event "Scan Bus": Value Change {
            n139 = event-data() -> ("NewVal"=w283:bool)  [unwired: 1 in]
            n140 = Type Cast(type=u8[] [] ("Payload"), x=w283) -> (*(type *) &x=w293:u8[])
            n141 = Bundle By Name(cluster=T2 {"Command"="", "Payload"=[]} ("Request Data"), "Command"="Scan Bus", "Payload"=w293) -> (w291:T2)
            n142 = Not Equal To 0?(x=w284) -> (x != 0?=w292:bool)
            n143 = case shown="True" w292 {
              tunnel: [w295 w297] -> w287
              tunnel: [w294 w296] -> w286
              tunnel: w284 -> [w295 w300]
              tunnel: w285 -> [w294 w299]
              tunnel: w291 -> [_ w298]
              frame False {
              }
              frame True {
                n144 = call "OOBgRPCService Generic.vi"("error in"=w299, "Request Data"=w298, "gRPC ID"=w300) -> ("error out"=w296:errorcluster, "gRPC ID out"=w297:T4)  [unwired: 6 in, 1 out]
              }
            }
          }
          event "Send I2C Script": Value Change {
            n145 = event-data() -> ("NewVal"=w307:bool)  [unwired: 1 in]
            n146 = local read "CONFIG SCRIPT FILE PATH"() -> (w308:path)
            n147 = local read "CMPLX SCRIPT"() -> (w301:bool)
            n148 = Path To String(path=w308) -> (string=w309:string)
            n149 = Bundle("NewVal"=w307, w309, "CMPLX SCRIPT"=w301) -> (w306:T5)  [unwired: 1 in]
            n150 = Flatten To String(anything=w306, error in (no error)=w303) -> (data string=w305:string, error out=w302:errorcluster)  [unwired: 2 in, 1 out]
            n151 = String To Byte Array(string=w305) -> (unsigned byte array=w304:u8[])
            n152 = Bundle By Name(cluster=T2 {"Command"="", "Payload"=[]} ("Request Data"), "Command"="I2C Script", "Payload"=w304) -> (w315:T2)
            n153 = Not Equal To 0?(x=w310) -> (x != 0?=w316:bool)
            n154 = case shown="True" w316 {
              tunnel: [w318 w320] -> w312
              tunnel: [w317 w319] -> w311
              tunnel: w310 -> [w318 w323]
              tunnel: w302 -> [w317 w322]
              tunnel: w315 -> [_ w321]
              frame False {
              }
              frame True {
                n155 = call "OOBgRPCService Generic.vi"("error in"=w322, "Request Data"=w321, "gRPC ID"=w323) -> ("error out"=w319:errorcluster, "gRPC ID out"=w320:T4)  [unwired: 6 in, 1 out]
              }
            }
          }
          event "Send I2C CMD": Value Change {
            n156 = event-data() -> ("NewVal"=w333:bool)  [unwired: 1 in]
            n157 = local read "SLAVE ADDR."() -> (w327:u8)
            n158 = local read "REG. ADDR."() -> (w326:u16)
            n159 = local read "DATA"() -> (w325:u8)
            n160 = local read "R/W"() -> (w324:bool)
            n161 = Bundle("NewVal"=w333, "SLAVE ADDR."=w327, "REG. ADDR."=w326, "DATA"=w325, "R/W"=w324) -> (w332:T6)  [unwired: 1 in]
            n162 = Flatten To String(anything=w332, error in (no error)=w329) -> (data string=w331:string, error out=w328:errorcluster)  [unwired: 2 in, 1 out]
            n163 = String To Byte Array(string=w331) -> (unsigned byte array=w330:u8[])
            n164 = Bundle By Name(cluster=T2 {"Command"="", "Payload"=[]} ("Request Data"), "Command"="I2C CMD", "Payload"=w330) -> (w339:T2)
            n165 = Not Equal To 0?(x=w334) -> (x != 0?=w340:bool)
            n166 = case shown="True" w340 {
              tunnel: [w342 w344] -> w336
              tunnel: [w341 w343] -> w335
              tunnel: w334 -> [w342 w347]
              tunnel: w328 -> [w341 w346]
              tunnel: w339 -> [_ w345]
              frame False {
              }
              frame True {
                n167 = call "OOBgRPCService Generic.vi"("error in"=w346, "Request Data"=w345, "gRPC ID"=w347) -> ("error out"=w343:errorcluster, "gRPC ID out"=w344:T4)  [unwired: 6 in, 1 out]
              }
            }
          }
          event User Event {
            n168 = event-data() -> ("Exit"=w350:bool)  [unwired: 1 in]
          }
        }
      }
      frame Default {
        w351 = u32 1000  # milliseconds to wait
        # "This delay is add here, because there are edge cases where the top loop is not ready to detect this loop errros."
        n169 = call "Stall Data Flow.vim"("value in"=w354, "milliseconds to wait"=w351) -> ("value out"=w352:errorcluster)  [unwired: 1 out]
        n170 = call "Send Async Loop Error.vi"("error in (no error)"=w352, "Measurement UI Queue"=w353) -> ()  [unwired: 9 in, 1 out]
      }
      frame Error {
        n171 = Unbundle By Name(w358) -> ("Status"=w361:refnum<vi>)
        n172 = Unbundle By Name(w358) -> ("RUNNING"=w359:refnum<vi>)
        n173 = local read "OOB gRPC Port"() -> (w366:i32)
        n174 = call "Update Running LED.vi"("RUNNING Ref"=w359, "Value"=FALSE) -> ()  [unwired: 9 in, 1 out]
        n175 = Equal?(x=w366, y=-1 ("x")) -> (x = y?=w364:bool)
        n176 = case shown="False" w364 {
          tunnel: w366 -> [w368 _]
          tunnel: [w367 "OOB gRPC server side Error.\nMeasrement Logic didn't get the gRPC port from OOB server.\nRestart the plugin." ("Status")] -> w360
          frame False {
            # "triggers event"
            n177 = disable-structure shown="Enabled" {
              disable-tunnel: ["OOB gRPC Disconnted!\nReconnecting.." ("Status") "Stopped" ("Status")] -> w367
              frame Disabled {
              }
              frame Enabled {
              }
            }
            n178 = property on="OOB gRPC Port" class="DigNum (strict)"("Val(Sgnl)"=w368) -> ()  [unwired: 2 in, 2 out]
          }
          frame True {
          }
        }
        n179 = call "Update Status.vi"("Value"=w360, "Status Ref"=w361) -> ()  [unwired: 9 in, 1 out]
      }
    }
  }
  n180 = while {
    tunnel: w3 -> [w378]
    tunnel: w16 -> [w377]
    tunnel: w7 -> [w374]
    tunnel: [w373] -> w4
    tunnel: w2 -> [w372]
    stop <- w379 stop-if-true
    # "UI events are hanlded in this loop, because handling them in the top loop while the plugin is running in IS, makes UI laggy."
    n181 = event shown="[3] \"HELP\": Value Change" {
      selector: w378 -> [_ _ _ _ _]
      dyn-events: _ -> [_ _ _ _ _]
      timeout: 100 -> [_ _ _ _ _]
      tunnel: [_ _ _ _ w420] -> w379
      tunnel: w377 -> [w385 w401 w409 _ _]
      tunnel: w374 -> [_ w399 _ _ _]
      tunnel: [w384 w398 w407 w419 _] -> w375
      tunnel: w372 -> [w380 _ _ w418 _]
      event Timeout {
        # "Dequeuing Buffer in this loop, to make it separate from the other loops' execution times, also to not add another loop just for this and make block diagram larger."
        # "Dequeues Buffer if not Paused"
        n182 = event-data() -> ()  [unwired: 1 in, 1 out]
        n183 = Unbundle By Name(w385) -> ("Status"=w381:refnum<vi>, "# TXNS IN TABLE"=w388:refnum<vi>, "MONITOR TABLE"=w387:refnum<vi>, "PauseResume"=w386:refnum<vi>)
        n184 = call-poly "Table Buffer.vi"("error in (no error)"=w380) -> ("error out"=w383:errorcluster, "# Elements in Buffer"=w382:i32)  [unwired: 8 in, 1 out]
        n185 = for {
          N: w382 -> [_]
          tunnel: w388 -> [w397]
          tunnel: w387 -> [w396]
          tunnel: w386 -> [w395]
          shift-right: [w390] -> w384
          shift-left: w383 -> [w391]
          tunnel: w381 -> [w389]
          stop <- w390 stop-if-true
          w394 = 10000  # Txns Limit
          n186 = call "Pause I2C Data.vi"("error in (no error)"=w391, "PauseResume Ref"=w395) -> ("error out"=w392:errorcluster, "I2C Data"=w393:string[][])  [unwired: 8 in]
          n187 = call "Update I2C Monitor Table.vi"("Status Ref"=w389, "Transactions Limit (10k)"=w394, "# TXNS IN TABLE Ref"=w397, "error in (no error)"=w392, "I2C Data in"=w393, "I2C Table Ref"=w396) -> ("error out"=w390:errorcluster)  [unwired: 5 in]
        }
      }
      event "Save CSV": Value Change {
        n188 = event-data() -> ("NewVal"=w400:bool)  [unwired: 1 in]
        n189 = case shown="True" w400 {
          tunnel: w401 -> [_ w404]
          tunnel: w399 -> [_ w403]
          tunnel: [_ w402] -> w398
          frame False {
          }
          frame True {
            n190 = Unbundle By Name(w404) -> ("CSV FILE PATH"=w406:refnum<vi>, "MONITOR TABLE"=w405:refnum<vi>)
            n191 = call "Save CSV (Async).vi"("CSV File Ref"=w406, "MONITOR TABLE Ref"=w405, "Measurement UI Queue"=w403) -> ("error out"=w402:errorcluster)  [unwired: 8 in]
          }
        }
      }
      event "Clear": Value Change {
        n192 = event-data() -> ("NewVal"=w408:bool)  [unwired: 1 in]
        n193 = case shown="True" w408 {
          tunnel: w409 -> [_ w415]
          tunnel: [_ w410] -> w407
          frame False {
          }
          frame True {
            n194 = Unbundle By Name(w415) -> ("Status"=w412:refnum<vi>, "# TXNS IN TABLE"=w413:refnum<vi>, "MONITOR TABLE"=w414:refnum<vi>)
            n195 = call "Clear I2C Monitor Table.vi"("# TXNS IN TABLE Ref"=w413, "I2C Table Ref"=w414) -> ("error out"=w411:errorcluster)  [unwired: 9 in]
            n196 = call "Update Status.vi"("error in (no error)"=w411, "Status Ref"=w412) -> ("error out"=w410:errorcluster)  [unwired: 9 in]
          }
        }
      }
      event "HELP": Value Change {
        n197 = event-data() -> ("NewVal"=w416:bool)  [unwired: 1 in]
        n198 = call "Open Help PDF.vi"("error in"=w418, "NewVal"=w416, "Path after documentation"=path "I2C Capture Plugin.pdf") -> ("error out"=w419:errorcluster)  [unwired: 8 in]
      }
      event User Event {
        n199 = event-data() -> ("Exit"=w420:bool)  [unwired: 1 in]
      }
    }
    n200 = call "Send Async Loop Error.vi"("error in (no error)"=w375, "Measurement UI Queue"=w374) -> ("error out"=w373:errorcluster)  [unwired: 9 in]
  }
  n201 = flat-sequence {
    tunnel: w3 -> [w422]
    tunnel: w4 -> [w421]
    frame #0 {
      n202 = Unregister For Events(event registration refnum=w422, error in=w421) -> ()  [unwired: 1 out]
    }
  }
  n203 = call "Destroy Client.vi"("gRPC ID"=w33) -> ("error out"=w5:errorcluster)  [unwired: 10 in]
  n204 = flat-sequence {
    tunnel: w20 -> [w423]
    tunnel: w5 -> [_]
    frame #0 {
      n205 = Unregister For Events(event registration refnum=w423) -> ()  [unwired: 1 in, 1 out]
    }
  }
